vi "Create.vi"(8 "error in (no error)":errorcluster) -> (0 "error out":errorcluster, 3 "Mock Class Generator out":refnum<class "Mock IPython Caller.lvclass">)   [LabVIEW 2026, in "Mock IPython Caller.lvclass"]
doc: "Create an instance of the mock class."
uses:
  Mock IPython Caller.lvclass
  Mock IPython Caller.lvclass/Mock IPython Caller.ctl
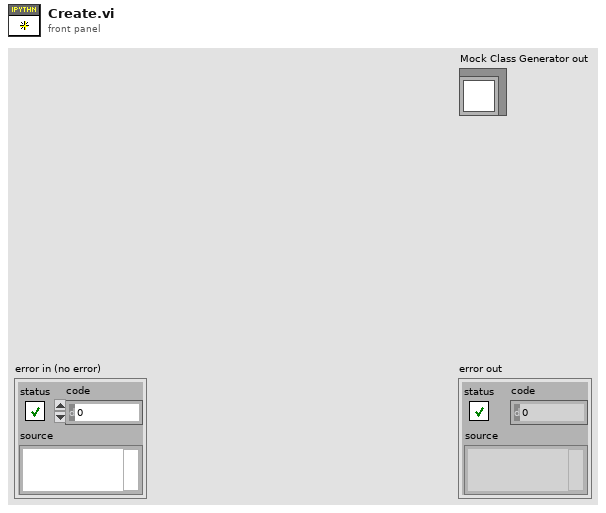
[diagram p1: front panel]
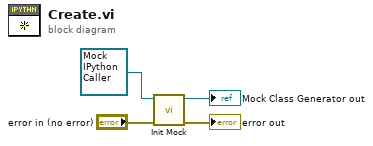
[diagram p0: block diagram]
diagram:
  n1 = call-dynamic "Init Mock.vi"("error in (no error)"="error in (no error)", "Mock In"=refnum<class "Mock IPython Caller.lvclass"> refnum ("Mock in")) -> ("error out"=→"error out":errorcluster, "Mock Out"=→"Mock Class Generator out":refnum<class "Mock IPython Caller.lvclass">)  [unwired: 8 in]
